vi "Add Link Button.vi"(8 "error in (no error)":errorcluster, 9 "URl":string, 10 "content":string, 11 "reference":refnum<k24>) -> (0 "error out":errorcluster, 3 "reference out":refnum<k24>)   [LabVIEW 2026, in "ToastNotification.lvlib" / "Toast Native.lvlib"]
doc: "Adds a protocol-activation button to a borrowed Microsoft.Toolkit.Uwp.Notifications.ToastContentBuilder using AddButton(String content, ToastActivationType activationType, String arguments). activationType is fixed to Protocol; URl is passed directly as the arguments string. Clicking the button asks Windows to open the URI with its associated application, rather than delivering this button action to the LabVIEW activation handler. No System.Uri or separate ToastButton handle is acquired by this VI. reference out aliases the borrowed builder; this VI does not close it. URL validation and native errors are delegated to the toolkit and Windows."
uses:
  Toast Native.lvlib
  C:/Users/loicw/Documents/LabVIEW/ToastNotifications/Sources/bins/Microsoft.Toolkit.Uwp.Notifications.dll
  bins/Microsoft.Toolkit.Uwp.Notifications.dll
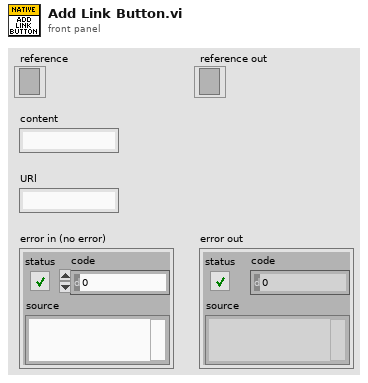
[diagram p1: front panel]
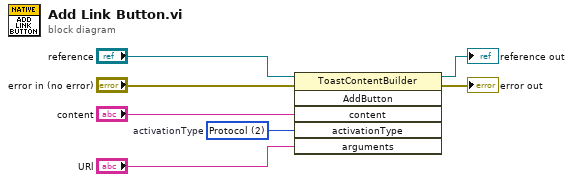
[diagram p0: block diagram]
diagram:
  w2 = 2 items=["Foreground", "Background", "Protocol"]  # activationType
  n1 = invoke class="ToastContentBuilder" method="AddButton"(reference="reference", error in="error in (no error)", "content"="content", "activationType"=w2, "arguments"="URl") -> (reference out=→"reference out":refnum<k24>, error out=→"error out":errorcluster)  [unwired: 1 in, 4 out]
